vi "Read User Timestamps FIFO.vi"(8 "error in (no error)":errorcluster, 11 "FPGA Ref in":refnum<k20>) -> (0 "error out":errorcluster, 2 "Data":u64[](array[numeric]), 3 "FPGA Ref out":refnum<k20>, 5 "Elements Remaining":u32)   [LabVIEW 2025, in "I2C Bus Monitor.lvclass"]
uses:
  I2C Bus Monitor.lvclass
  <vilib>/Utility/error.llb/Error Cluster From Error Code.vi
  <vilib>/rvi/errors/niLvFpgaAdjustHostInterfaceError.vi
  <vilib>/rvi/interface/nirviMethod/nirviMethod.xnode
  I2C Bus Monitor.lvclass/I2C Bus Monitor.ctl
  <vilib>/FPGAPlugInAG/Dynamic/niLvFpga_ReadFifo_Dynamic.vi
  <vilib>/rvi/errors/niLvFpgaMergeErrorWithErrorCode.vi
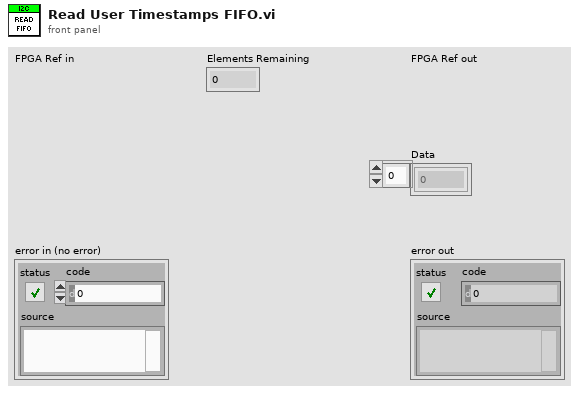
[diagram p1: front panel]
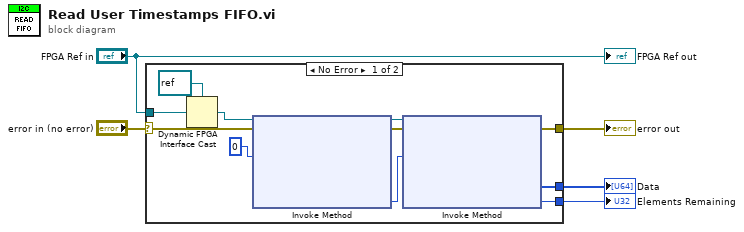
[diagram p0: block diagram]
diagram:
  n1 = case shown="No Error" "error in (no error)" {
    selector: "error in (no error)" -> [w15 w17]
    tunnel: [w16 w17] -> w5
    tunnel: [w11 _] -> w3
    tunnel: [w9 _] -> w2
    tunnel: "FPGA Ref in" -> [w6 _]
    frame No Error {
      n2 = Dynamic FPGA Interface Cast(Session In=refnum<k20> refnum ("FPGA VI Reference Out"), Type=w6) -> (Session Out=w13:refnum<k20>)
      n3 = xnode "Invoke Method"("FPGA VI Reference In"=w13, "error in"=w15, "Number of Elements"=u32 0) -> ("FPGA VI Reference Out"=w7:refnum<k20>, "error out"=w8:errorcluster, "Elements Remaining"=w10:u32)  [unwired: 1 in, 1 out]
      n4 = xnode "Invoke Method"("FPGA VI Reference In"=w7, "error in"=w8, "Number of Elements"=w10) -> ("error out"=w16:errorcluster, "Data"=w11:u64[], "Elements Remaining"=w9:u32)  [unwired: 1 in, 1 out]
    }
    frame Error {
    }
  }
  "error out" <- w5
  "Data" <- w3
  "Elements Remaining" <- w2
  "FPGA Ref out" <- "FPGA Ref in"
